vi "[ce] Index Range to Flattened String.vi"(11 "Index Range":cluster{"Initial index":i32, "Final index":i32}) -> (3 "Flattened string":string)   [LabVIEW 2021]
doc: "::: CalcExpress Toolkit :::\nCopyright (c) 2000-2026 Konstantin Shifershteyn. All rights reserved."
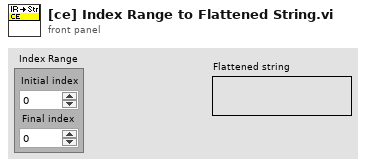
[diagram p1: front panel]
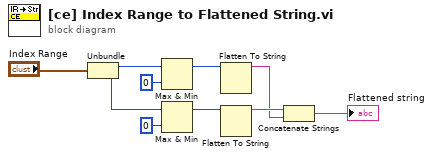
[diagram p0: block diagram]
diagram:
  n1 = Unbundle("Index Range") -> ("Initial index"=w10:i32, "Final index"=w5:i32)
  n2 = Max & Min(x=w10, y=0) -> (max(x,y)=w8:i32)  [unwired: 1 out]
  n3 = Max & Min(x=w5, y=0) -> (max(x,y)=w4:i32)  [unwired: 1 out]
  n4 = Flatten To String(anything=w8) -> (data string=w2:string)  [unwired: 3 in, 2 out]
  n5 = Flatten To String(anything=w4) -> (data string=w3:string)  [unwired: 3 in, 2 out]
  n6 = Concatenate Strings(w3, w2) -> (→"Flattened string":string)
